vi "test_tool_with_progress.vi"(8 "error in":errorcluster) -> (0 "error out":errorcluster, 3 "text":string)   [LabVIEW 2020, in "Conformance MCP Server.lvlib"]
doc: "Conformance fixture (scenario tools-call-with-progress). Takes no arguments. Reports the progress 0, 50 and 100 of total 100 with Report Progress.vi, 50 ms apart, then returns the text \"progress done\". A client that sends a progressToken receives three notifications/progress before the result."
uses:
  Conformance MCP Server.lvlib
  src/MCP Server/MCP Server.lvlib
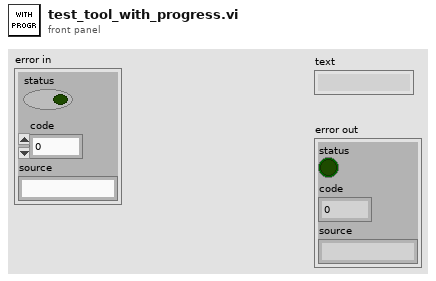
[diagram p1: front panel]
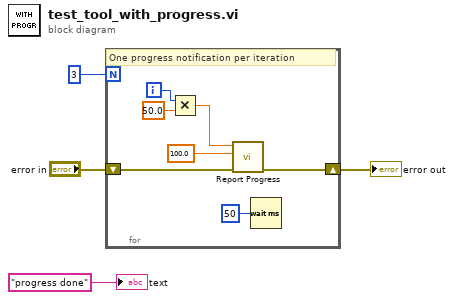
[diagram p0: block diagram]
diagram:
  n1 = for {
    N: 3 ("count") -> [_]
    shift-right: [w10] -> w3
    shift-left: "error in" -> [w11]
    i -> [w5]
    # "One progress notification per iteration"
    n2 = Multiply(x=w5, y=50.0 ("step")) -> (x*y=w9:dbl)
    n3 = call "Report Progress.vi"("error in"=w11, "total"=100.0, "progress"=w9) -> ("error out"=w10:errorcluster)  [unwired: 7 in, 1 out]
    n4 = Wait (ms)(milliseconds to wait=u32 50) -> ()  [unwired: 1 out]
  }
  "error out" <- w3
  "text" <- "progress done" ("text")
